vi "WriteFLBuffer.vi"(6 "error in":errorcluster, 7 "string in":string, 9 "connection ID in":refnum<k5>) -> (0 "error out":errorcluster, 3 "connection ID out":refnum<k5>)   [LabVIEW 2014]
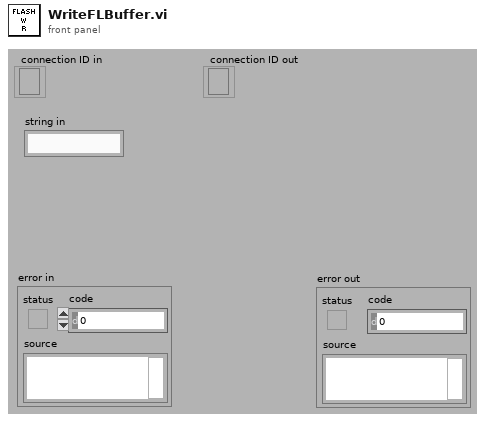
[diagram p1: front panel]
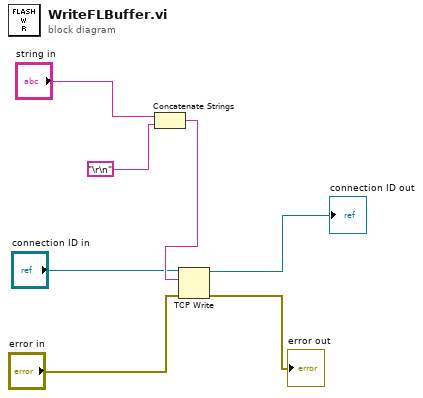
[diagram p0: block diagram]
diagram:
  n1 = Concatenate Strings("string in", "\r\n") -> (w7:string)
  n2 = TCP Write(connection ID="connection ID in", data in=w7, error in (no error)="error in") -> (connection ID out=→"connection ID out":refnum<k5>, error out=→"error out":errorcluster)  [unwired: 1 in, 1 out]
